vi "query Limit Line Pass Fail.vi"(8 "error in (no error)":errorcluster, 10 "Limit Line Index":i32=1 min=1 max=8, 11 "Keysight 9020A in":refnum<class "Keysight 9020A.lvclass">) -> (0 "error out":errorcluster, 2 "Pass?":bool, 3 "Keysight 9020A out":refnum<class "Keysight 9020A.lvclass">)   [LabVIEW 2023, in "Spectrum Analyzer.lvlib" / "Keysight 9020A.lvclass"]
uses:
  Keysight 9020A.lvclass
  Keysight 9020A.lvclass/Keysight 9020A.ctl
  Spectrum Analyzer.lvlib
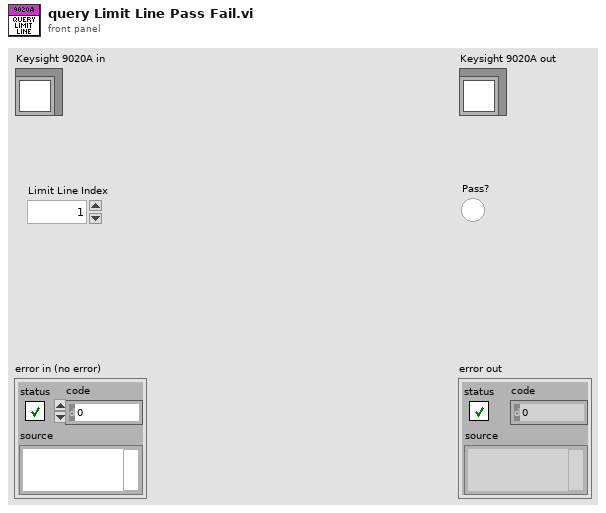
[diagram p1: front panel]
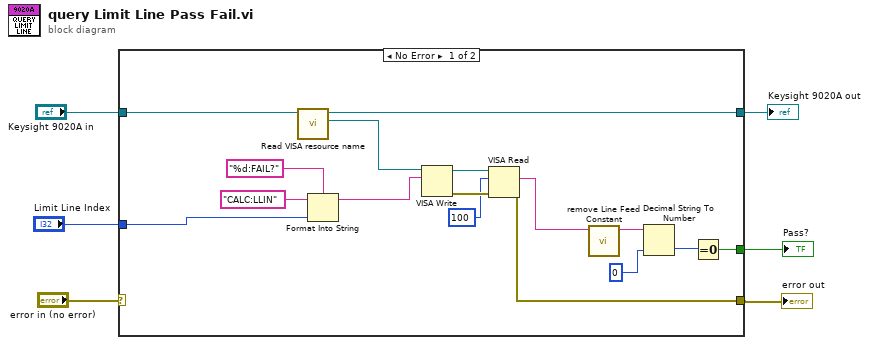
[diagram p0: block diagram]
diagram:
  n1 = case shown="No Error" "error in (no error)" {
    selector: "error in (no error)" -> [_ w23]
    tunnel: "Keysight 9020A in" -> [w14 w24]
    tunnel: [w22 w24] -> w5
    tunnel: [w16 w23] -> w3
    tunnel: "Limit Line Index" -> [w11 _]
    tunnel: [w8 _] -> w1
    frame No Error {
      n2 = call "Read VISA resource name.vi"("Keysight 9020A in"=w14) -> ("VISA resource name"=w7:refnum<visa-resource-name>, "Keysight 9020A out"=w22:refnum<class "Keysight 9020A.lvclass">)  [unwired: 8 in, 1 out]
      n3 = Format Into String(format string="%d:FAIL?", initial string="CALC:LLIN", w11) -> (resulting string=w10:string)  [unwired: 1 in, 1 out]
      n4 = VISA Write(VISA resource name=w7, write buffer=w10) -> (VISA resource name out=w21:refnum<visa-resource-name>, error out=w20:errorcluster)  [unwired: 1 in, 1 out]
      n5 = VISA Read(VISA resource name=w21, byte count=u32 100, error in (no error)=w20) -> (read buffer=w18:string, error out=w16:errorcluster)  [unwired: 2 out]
      n6 = call "remove Line Feed Constant.vi"("Input String"=w18) -> ("Line Feed Removed String"=w17:string)  [unwired: 10 in]
      n7 = Decimal String To Number(string=w17, default (0L)=u32 0) -> (number=w9:u32)  [unwired: 1 in, 1 out]
      n8 = Equal To 0?(x=w9) -> (x = 0?=w8:bool)
    }
    frame Error {
    }
  }
  "error out" <- w3
  "Keysight 9020A out" <- w5
  "Pass?" <- w1
